vi "Registry Global.vi"() -> ()   [LabVIEW 2018, in "GLog.lvlib" / "Registry.lvlib"]
uses:
  Registry.lvlib
panel:
  in  "registry vi ref":refnum<vi>
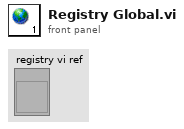
[diagram p1: front panel]
diagram:
